vi "LabVIEW.FGV.Store_ID.vi"(0 "ID In":string, 1 "Command":enum16{"clear", "write", "read"}(ring), 5 "Step IDs in[]":string[](array[string]), 7 "Fertigmeldung in[]":string[](array[string]), 9 "Step types in[]":string[](array[string]), 11 "error in (no error)":errorcluster caption="Fehler (Eingang, kein Fehler)", 12 "File Name In":string) -> (4 "ID Out":string, 6 "Step IDs out[]":string[](array[string]), 8 "Fertigmeldung out[]":string[](array[string]), 10 "Step types out[]":string[](array[string]), 14 "File Name Out":string, 15 "error out":errorcluster caption="Fehler (Ausgang)")   [LabVIEW 2019]
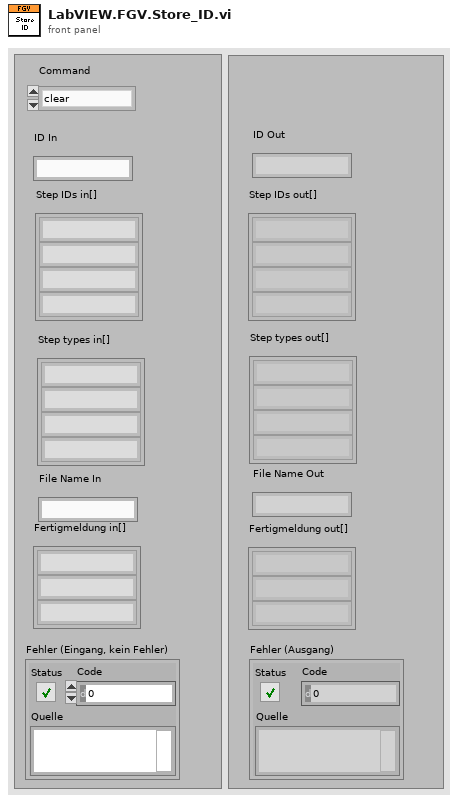
[diagram p1: front panel]
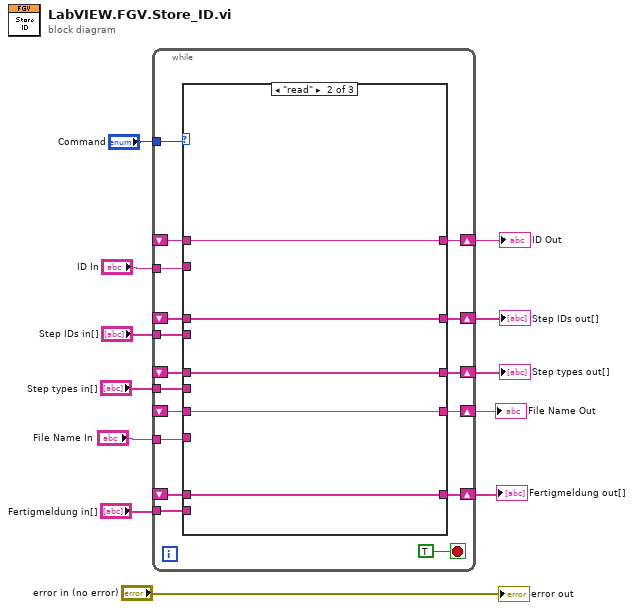
[diagram p0: block diagram]
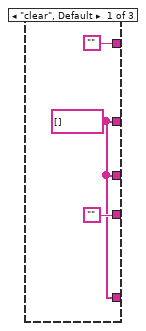
[diagram p2: hidden frame]
diagram:
  n1 = while {
    tunnel: "Command" -> [w28]
    shift-right: [w27] -> w10
    shift-left: _ -> [w25]
    tunnel: "ID In" -> [w26]
    tunnel: "Step IDs in[]" -> [w24]
    shift-right: [w23] -> w7
    shift-left: _ -> [w22]
    tunnel: "Step types in[]" -> [w19]
    shift-right: [w20] -> w6
    shift-left: _ -> [w21]
    shift-right: [w16] -> w3
    shift-left: _ -> [w18]
    tunnel: "File Name In" -> [w17]
    tunnel: "Fertigmeldung in[]" -> [w13]
    shift-right: [w14] -> w2
    shift-left: _ -> [w15]
    stop <- TRUE stop-if-true
    n2 = case shown="\"read\"" w28 {
      tunnel: w26 -> [_ _ w42]
      tunnel: ["" w37 w42] -> w27
      tunnel: w25 -> [_ w37 _]
      tunnel: w24 -> [_ _ w41]
      tunnel: [w30 w36 w41] -> w23
      tunnel: w22 -> [_ w36 _]
      tunnel: w19 -> [_ _ w40]
      tunnel: [w30 w35 w40] -> w20
      tunnel: w21 -> [_ w35 _]
      tunnel: w17 -> [_ _ w39]
      tunnel: ["" w34 w39] -> w16
      tunnel: w18 -> [_ w34 _]
      tunnel: w13 -> [_ _ w38]
      tunnel: [w30 w33 w38] -> w14
      tunnel: w15 -> [_ w33 _]
      frame "clear", Default {
        w30 = string[] [] ("Step IDs in[]")
      }
      frame "read" {
      }
      frame "write" {
      }
    }
  }
  "ID Out" <- w10
  "Step IDs out[]" <- w7
  "Step types out[]" <- w6
  "File Name Out" <- w3
  "Fertigmeldung out[]" <- w2
  "error out" <- "error in (no error)"
